vi "Own20261013_CreateClass.vi"() -> ()   [LabVIEW 2024]
uses:
  <resource>/Framework/Providers/AddClass/Add Class.lvlib
panel:
  out "error out":errorcluster caption="错误输出"
  in  "Parent Interfaces":refnum<vi>[](array[refnum])
  in  "Parent Class":refnum<vi>
  in  "error in":errorcluster
  in  "New Class Owner":refnum<vi>
  in  "Class Path":path
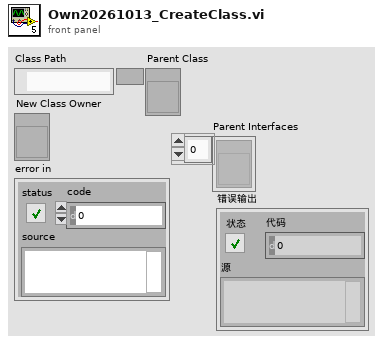
[diagram p1: front panel]
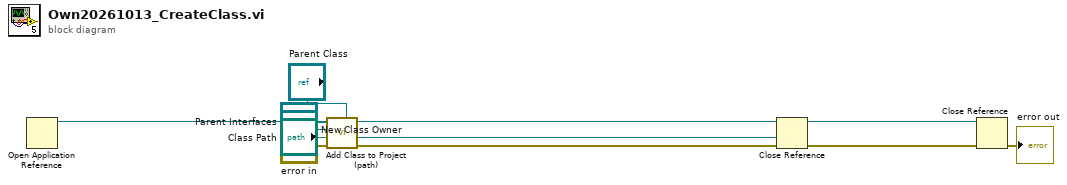
[diagram p0: block diagram]
diagram:
  n1 = Open Application Reference() -> (3:w5:refnum<vi>)  [unwired: 4 in, 1 out]
  n2 = call <resource>:"Add Class to Project (path).vi"("Parent Class"="Parent Class", "Application"=w5, "error in"="error in", "Class Path"="Class Path", "New Class Owner"="New Class Owner", "Parent Interfaces"="Parent Interfaces") -> ("error out"=w3:errorcluster, "Class"=w4:refnum<vi>)  [unwired: 4 in]
  n3 = Close Reference(reference=w4, error in (no error)=w3) -> (error out=w2:errorcluster)
  n4 = Close Reference(reference=w5, error in (no error)=w2) -> (error out=→"error out":errorcluster)
